vi "set TXP Threshold Type.vi"(8 "error in (no error)":errorcluster, 10 "Type":enum16{"Absolute", "Relative"}(ring), 11 "Keysight 9020A in":refnum<class "Keysight 9020A.lvclass">) -> (0 "error out":errorcluster, 3 "Keysight 9020A out":refnum<class "Keysight 9020A.lvclass">)   [LabVIEW 2023, in "Spectrum Analyzer.lvlib" / "Keysight 9020A.lvclass"]
uses:
  Keysight 9020A.lvclass
  Keysight 9020A.lvclass/Keysight 9020A.ctl
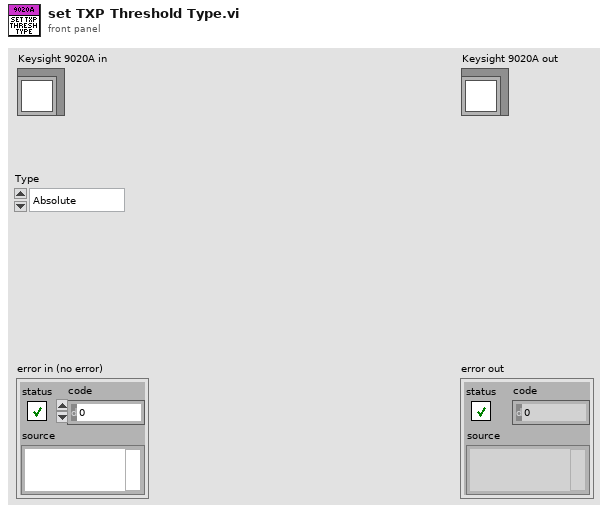
[diagram p1: front panel]
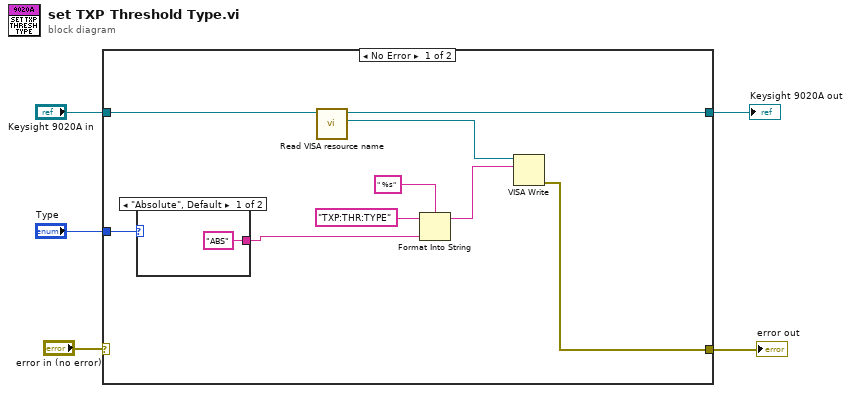
[diagram p0: block diagram]
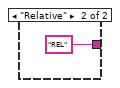
[diagram p2: hidden frame]
diagram:
  n1 = case shown="No Error" "error in (no error)" {
    selector: "error in (no error)" -> [_ w17]
    tunnel: "Keysight 9020A in" -> [w9 w18]
    tunnel: [w14 w18] -> w4
    tunnel: [w10 w17] -> w1
    tunnel: "Type" -> [w8 _]
    frame No Error {
      n2 = case shown="\"Absolute\", Default" w8 {
        tunnel: ["ABS" "REL"] -> w6
        frame "Absolute", Default {
        }
        frame "Relative" {
        }
      }
      n3 = call "Read VISA resource name.vi"("Keysight 9020A in"=w9) -> ("VISA resource name"=w12:refnum<visa-resource-name>, "Keysight 9020A out"=w14:refnum<class "Keysight 9020A.lvclass">)  [unwired: 8 in, 1 out]
      n4 = Format Into String(format string=" %s", initial string="TXP:THR:TYPE" ("string"), w6) -> (resulting string=w11:string)  [unwired: 1 in, 1 out]
      n5 = VISA Write(VISA resource name=w12, write buffer=w11) -> (error out=w10:errorcluster)  [unwired: 1 in, 2 out]
    }
    frame Error {
    }
  }
  "error out" <- w1
  "Keysight 9020A out" <- w4
